vi "Signal FPGA to start acquisition.vi"(8 "error in (no error)":errorcluster, 10 "Logging queue element":T3={"Imaging Protocol"=enum."Live Imaging", "Number of Trials"=0, "Frame Size"=512, "# Averaged frames"=0, "Dwell time (us)"=0.0, "Index of Z-plane"=0, "Timelapse?"=FALSE, "Logging process is active"=FALSE, "Speed logging enabled"=FALSE, "tdms file ref"=refnum, "path"=path "", "Trial Number"=0, "Expected # points acquired"=FALSE, "Manually stopped"=FALSE, "Last trial"=FALSE, "Ch0 data"=[], "Ch1 data"=[], "Ref Data"=[], "Ref Frame Time"=[], "Image Time"=[], "Continuous Time"=[], "Ref X Length"=0, "Ref Y Length"=0, "# Ref Averaged frames"=0, "Ref Dwell time (us)"=0.0, "Points acquired"={"Ch0 last trial"=0, "Ch1 last trial"=0, "All trials"=0}, "HW Timings File"=refnum} {"Ref Dwell time (us)" format="%#.6g"; "Frame Size" items=["100X100"=100, "128X128"=128, "200X200"=200, "256X256"=256, "512X512"=512, "1024x1024"=1024, "2048x2048"=2048]; "Dwell time (us)" format="%#.6g"}, 11 "FPGA VI Ref":T2) -> (0 "error out":errorcluster, 3 "FPGA VI Reference Out":T2)   [LabVIEW 2020]
uses:
  RIG-SPECIFIC FILES/FPGA Refs/FPGA Ref.ctl
  Typedefs/Logging queue element.ctl
  Typedefs/Imaging Protocols enum.ctl
  Typedefs/Frame Size.ctl
  Typedefs/Acquired points count.ctl
  <vilib>/Utility/error.llb/Error Cluster From Error Code.vi
  <vilib>/rvi/errors/niLvFpgaAdjustHostInterfaceError.vi
  Global Variables/General Globals.vi
  <vilib>/rvi/interface/nirviReadWriteControl/nirviReadWriteControl.xnode
  NiFpgaLv.dll
  <vilib>/rvi/interface/Simulation/niFpgaSimulationCallBeginRW.vi
panel:
  out "Imaging Protocol":T1
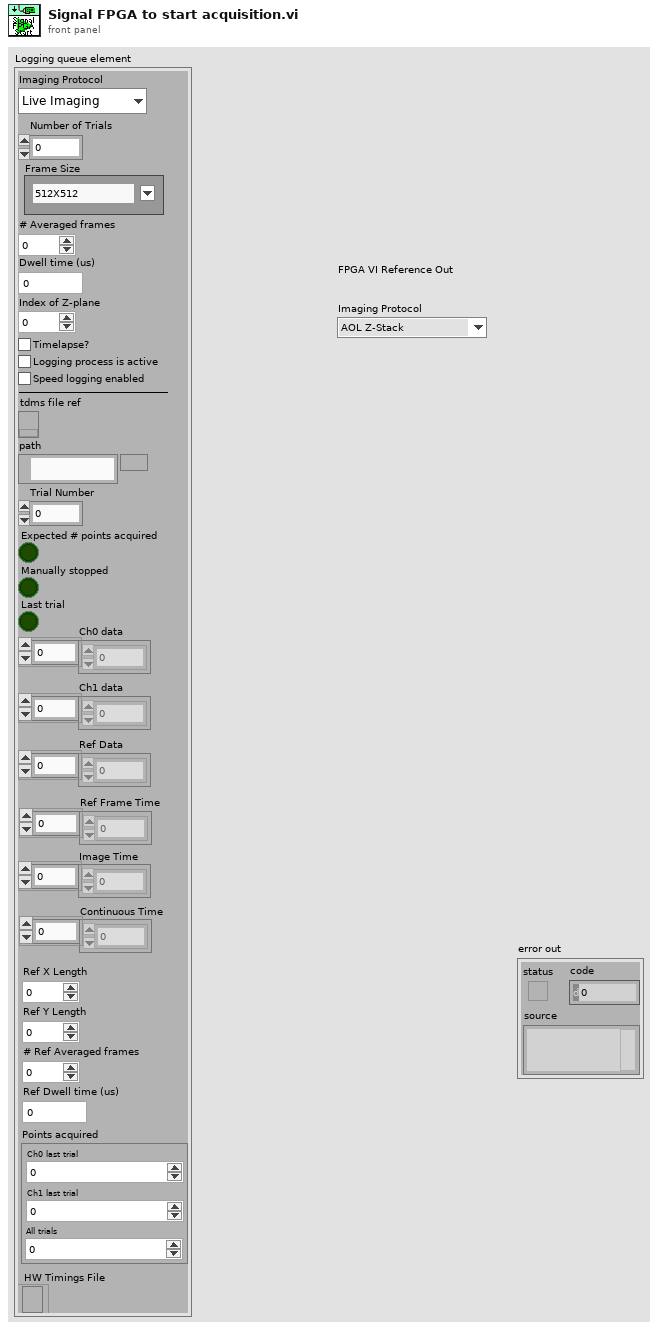
[diagram p1: front panel]
types:
  T1 = typedef "Imaging Protocols enum.ctl" = enum16{"AOL Z-Stack", "Motor Z Stack", "Parameter Sweep", "Functional Acquisition", "Single Plane Acquisition", "Volume Acquisition", "Live Imaging", "Live Plane Imaging", "Live Volume Imaging"}
  T2 = typedef "FPGA Ref.ctl" = refnum<k20>
  T3 = typedef "Logging queue element.ctl" = cluster{"Imaging Protocol":T1, "Number of Trials":u16, "Frame Size":T4, "# Averaged frames":u16, "Dwell time (us)":dbl, "Index of Z-plane":i32, "Timelapse?":bool, "Logging process is active":bool, "Speed logging enabled":bool, "tdms file ref":refnum<k34>, "path":path, "Trial Number":i32, "Expected # points acquired":bool, "Manually stopped":bool, "Last trial":bool, "Ch0 data":u32[], "Ch1 data":u32[], "Ref Data":u32[], "Ref Frame Time":u64[], "Image Time":u64[], "Continuous Time":u64[], "Ref X Length":u16, "Ref Y Length":u16, "# Ref Averaged frames":u16, "Ref Dwell time (us)":dbl, "Points acquired":T5, "HW Timings File":refnum<file>}
  T4 = typedef "Frame Size.ctl" = u16
  T5 = typedef "Acquired points count.ctl" = cluster{"Ch0 last trial":u64, "Ch1 last trial":u64, "All trials":u64}
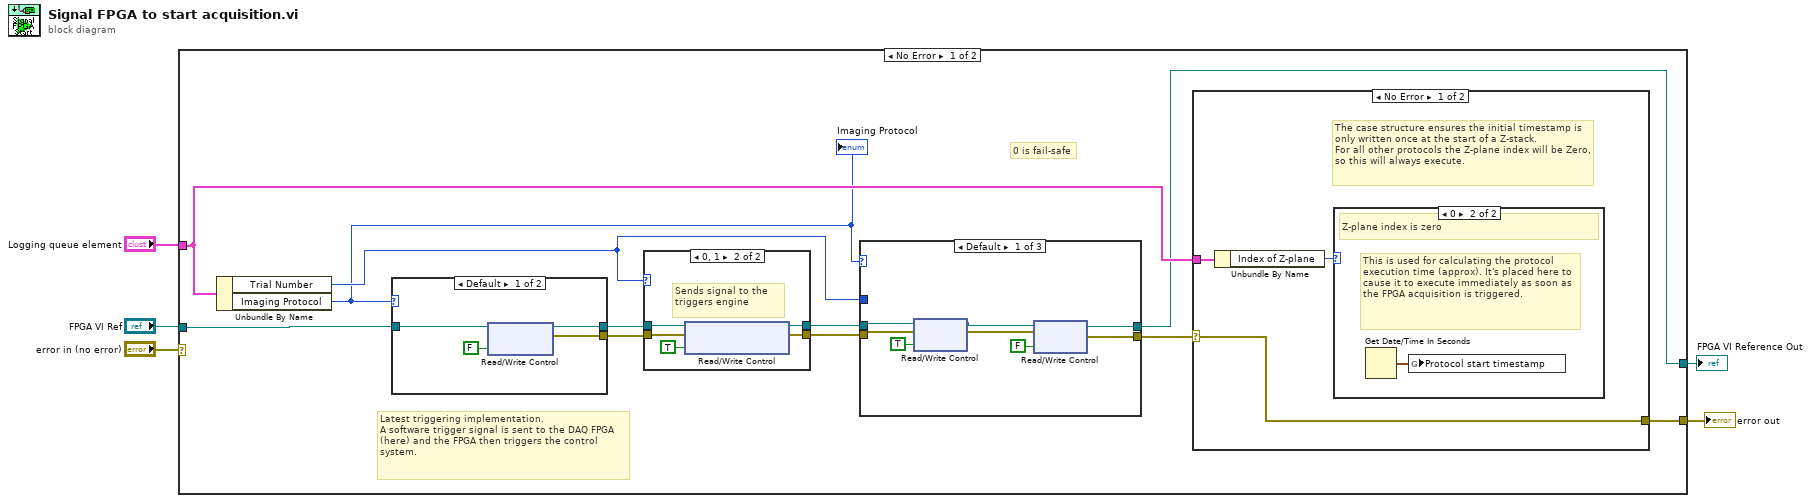
[diagram p0: block diagram]
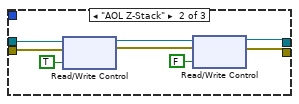
[diagram p2: hidden frame]
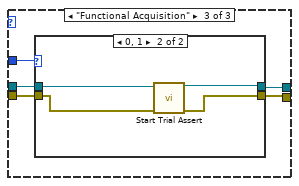
[diagram p3: hidden frame]
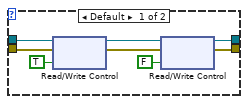
[diagram p4: hidden frame]
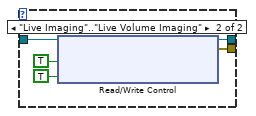
[diagram p8: hidden frame]
diagram:
  n1 = case shown="No Error" "error in (no error)" {
    selector: "error in (no error)" -> [_ w72]
    tunnel: [w15 w72] -> w5
    tunnel: "FPGA VI Ref" -> [w16 w71]
    tunnel: "Logging queue element" -> [w14 _]
    tunnel: [w6 w71] -> w1
    frame No Error {
      # "0 is fail-safe"
      # "Latest triggering implementation.\nA software trigger signal is sent to the DAQ FPGA (here) and the FPGA then triggers the control system."
      n2 = Unbundle By Name(w14) -> ("Trial Number"=w11:i32, "Imaging Protocol"=w8:T1)
      "Imaging Protocol" <- w8
      n3 = case shown="Default" w8 {
        tunnel: w16 -> [w64 w70]
        tunnel: [w63 w69] -> w13
        tunnel: [w62 w67] -> w12
        frame Default {
          n4 = xnode "Read/Write Control"("FPGA VI Reference In"=w64, "live_scan"=FALSE) -> ("FPGA VI Reference Out"=w63:T2, "error out"=w62:errorcluster)  [unwired: 1 in]
        }
        frame "Live Imaging".."Live Volume Imaging" {
          n5 = xnode "Read/Write Control"("FPGA VI Reference In"=w70, "live_scan"=TRUE, "live_scan (triggers module)"=TRUE) -> ("FPGA VI Reference Out"=w69:T2, "error out"=w67:errorcluster)  [unwired: 1 in]
        }
      }
      n6 = case shown="0, 1" w11 {
        tunnel: w12 -> [w51 w55]
        tunnel: [w51 w54] -> w9
        tunnel: w13 -> [w50 w53]
        tunnel: [w50 w52] -> w10
        frame Default {
        }
        frame 0, 1 {
          # "Sends signal to the triggers engine"
          n7 = xnode "Read/Write Control"("FPGA VI Reference In"=w53, "error in"=w55, "Experiment start"=TRUE ("start")) -> ("FPGA VI Reference Out"=w52:T2, "error out"=w54:errorcluster)
        }
      }
      n8 = case shown="Default" w8 {
        tunnel: w10 -> [w23 w30 w36]
        tunnel: w9 -> [w22 w31 w34]
        tunnel: [w18 w27 w35] -> w6
        tunnel: [w17 w26 w33] -> w7
        tunnel: w11 -> [_ _ w37]
        frame Default {
          n9 = xnode "Read/Write Control"("FPGA VI Reference In"=w23, "error in"=w22, "start"=TRUE) -> ("FPGA VI Reference Out"=w20:T2, "error out"=w19:errorcluster)
          n10 = xnode "Read/Write Control"("FPGA VI Reference In"=w20, "error in"=w19, "start"=FALSE) -> ("FPGA VI Reference Out"=w18:T2, "error out"=w17:errorcluster)
        }
        frame "AOL Z-Stack" {
          n11 = xnode "Read/Write Control"("FPGA VI Reference In"=w30, "error in"=w31, "start"=TRUE) -> ("FPGA VI Reference Out"=w29:T2, "error out"=w28:errorcluster)
          n12 = xnode "Read/Write Control"("FPGA VI Reference In"=w29, "error in"=w28, "start"=FALSE) -> ("FPGA VI Reference Out"=w27:T2, "error out"=w26:errorcluster)
        }
        frame "Functional Acquisition" {
          n13 = case shown="0, 1" w37 {
            tunnel: w36 -> [w44 w49]
            tunnel: [w41 w47] -> w35
            tunnel: w34 -> [w43 w48]
            tunnel: [w38 w46] -> w33
            frame Default {
              n14 = xnode "Read/Write Control"("FPGA VI Reference In"=w44, "error in"=w43, "start"=TRUE) -> ("FPGA VI Reference Out"=w40:T2, "error out"=w39:errorcluster)
              n15 = xnode "Read/Write Control"("FPGA VI Reference In"=w40, "error in"=w39, "start"=FALSE) -> ("FPGA VI Reference Out"=w41:T2, "error out"=w38:errorcluster)
            }
            frame 0, 1 {
              n16 = call "Start Trial Assert.vi"("error in"=w48, "FPGA VI Ref"=w49) -> ("error out"=w46:errorcluster, "FPGA VI Reference Out"=w47:T2)  [unwired: 8 in]
            }
          }
        }
      }
      n17 = case shown="No Error" w7 {
        selector: w7 -> [w59 w61]
        tunnel: [w59 w61] -> w15
        tunnel: w14 -> [w58 _]
        frame No Error {
          # "The case structure ensures the initial timestamp is only written once at the start of a Z-stack.\nFor all other protocols the Z-plane index will be Zero, so this will always execute."
          n18 = Unbundle By Name(w58) -> ("Index of Z-plane"=w57:i32)
          n19 = case shown="0" w57 {
            frame Default {
              # "Z-plane index is other than zero"
            }
            frame 0 {
              # "This is used for calculating the protocol execution time (approx). It's placed here to cause it to execute immediately as soon as the FPGA acquisition is triggered."
              # "Z-plane index is zero"
              n20 = Get Date/Time In Seconds() -> (seconds since 1Jan1904=w60:timestamp)
              n21 = global write "General Globals.vi" "Protocol start timestamp"(w60) -> ()
            }
          }
        }
        frame Error {
        }
      }
    }
    frame Error {
    }
  }
  "error out" <- w5
  "FPGA VI Reference Out" <- w1
